vi "Run Socket.vi"(8 "error in (no error)":errorcluster caption="에러 입력(에러 없음)", 11 "TCP Socket 입력":refnum<class "TCP Socket.lvclass">) -> (0 "error out":errorcluster caption="에러 출력", 3 "TCP Socket 출력":refnum<class "TCP Socket.lvclass">)   [LabVIEW 2023, in "TCP Socket.lvclass"]
uses:
  TCP Socket.lvclass
  TCP Socket.lvclass/TCP Socket.ctl
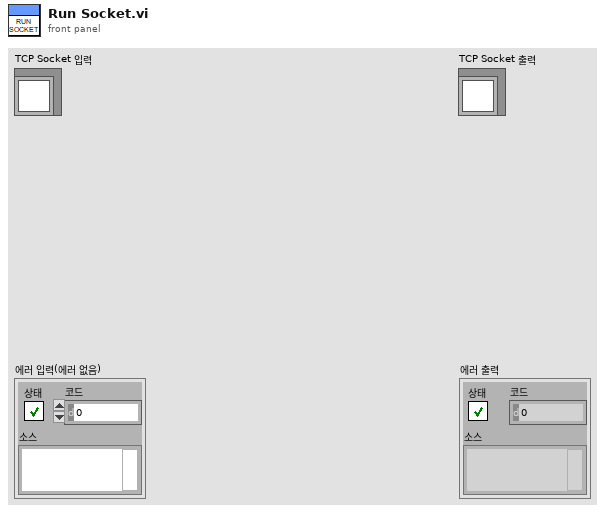
[diagram p1: front panel]
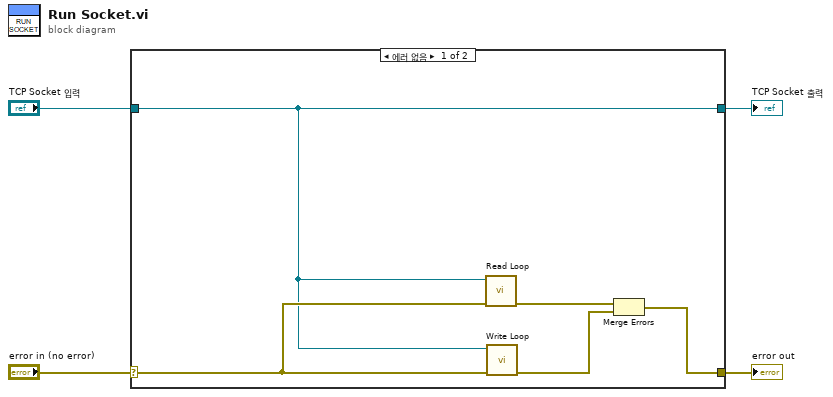
[diagram p0: block diagram]
diagram:
  n1 = case shown="에러 없음" "error in (no error)" {
    selector: "error in (no error)" -> [w9 w11]
    tunnel: [w8 w11] -> w3
    tunnel: [w7 w10] -> w1
    tunnel: "TCP Socket 입력" -> [w7 w10]
    frame No Error {
      n2 = call "Read Loop.vi"("error in (no error)"=w9, "TCP Socket 입력"=w7) -> ("error out"=w6:errorcluster)  [unwired: 8 in, 1 out]
      n3 = call "Write Loop.vi"("error in (no error)"=w9, "TCP Socket 입력"=w7) -> ("error out"=w5:errorcluster)  [unwired: 8 in, 1 out]
      n4 = Merge Errors(w6, w5) -> (w8:errorcluster)
    }
    frame Error {
    }
  }
  "error out" <- w3
  "TCP Socket 출력" <- w1
